vi "RDC-saltwater-generate_perm_from_freq.vi"(10 "Frequency":dbl[](array[numeric]), 11 "water Temp (25C) [10-40C]":dbl=25.0) -> (1 "Complex Perm":cluster{dbl[], cdb[]}, 2 "Imag Perm":cluster{dbl[], dbl[]}, 3 "Real Perm":cluster{dbl[], dbl[]}, 4 "Complex perm":cdb[](array[numeric]))   [LabVIEW 2020, in "RDC-Reflection_Data_Computation.lvlib"]
doc: "Generates the salt water model permittivity for the given frequency array at the given water temperature (10-40 C), using RDC-saltwater-generate_perm."
uses:
  RDC-Reflection_Data_Computation.lvlib
panel:
  out "size(s) 2":i32
  out "size(s)":i32
  out "loss":cluster{dbl[], dbl[]}(graph)
  out "perm":cluster{dbl[], dbl[]}(graph)
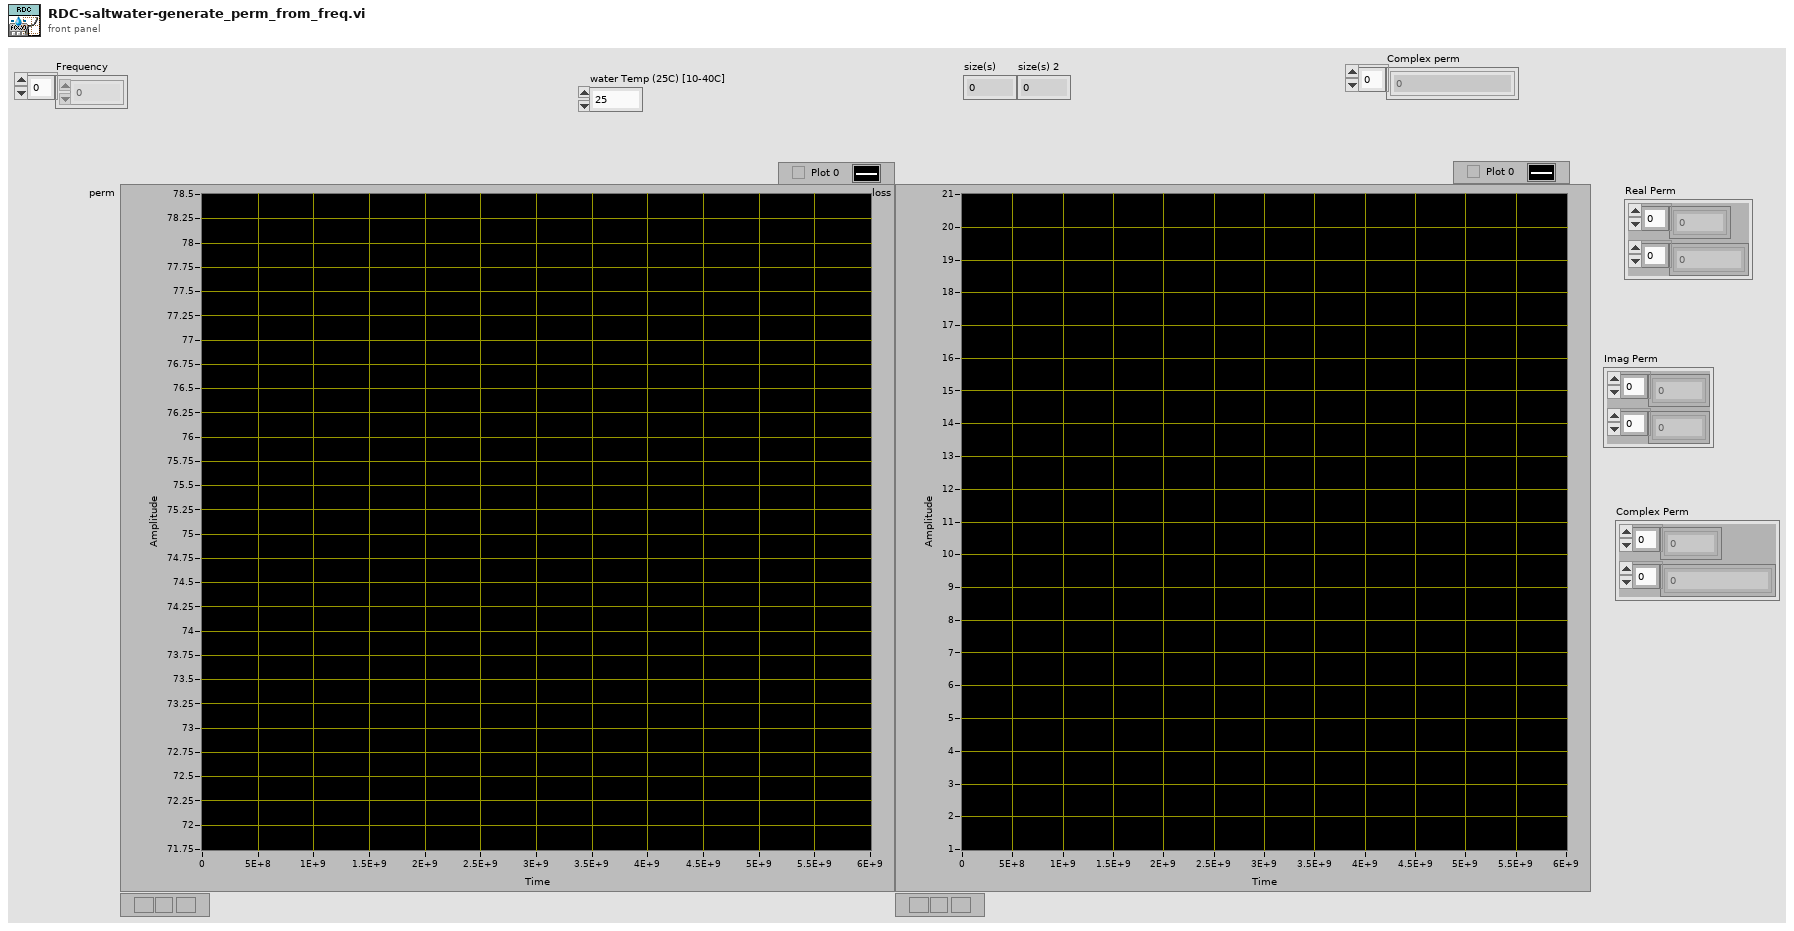
[diagram p1: front panel]
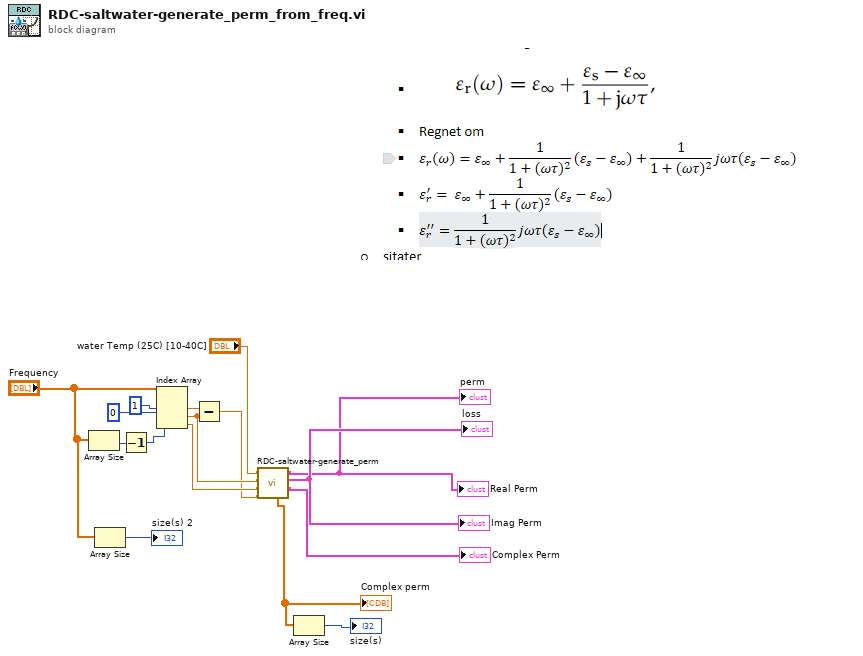
[diagram p0: block diagram]
diagram:
  n1 = Array Size(array="Frequency") -> (size(s)=w14:i32)
  n2 = Array Size(array="Frequency") -> (size(s)=→"size(s) 2":i32)
  n3 = Decrement(x=w14) -> (x-1=w13:i32)
  n4 = Index Array(array="Frequency", index #1=1 ("index"), index #2=0 ("index"), index #3=w13) -> (element #1=w12:dbl, element #2=w7:dbl, element #3=w6:dbl)
  n5 = Subtract(x=w12, y=w7) -> (x-y=w5:dbl)
  n6 = call "RDC-saltwater-generate_perm.vi"("Increment f (10MHz)"=w5, "Stop f (6GHz) 2"=w6, "Start f (300MHz)"=w7, "water Temp (25C) [10-40C]"="water Temp (25C) [10-40C]") -> ("Complex Perm"=→"Complex Perm":cluster{dbl[], cdb[]}, "Imag Perm"=→"Imag Perm" →"loss":cluster{dbl[], dbl[]}, "Real Perm"=→"Real Perm" →"perm":cluster{dbl[], dbl[]}, "Complex perm"=w4:cdb[])  [unwired: 3 in, 1 out]
  "Complex perm" <- w4
  n7 = Array Size(array=w4) -> (size(s)=→"size(s)":i32)
